vi "Remove Child.vi"(8 "error in (no error)":errorcluster, 10 "Child":refnum<data-value>, 11 "NodeRef In":refnum<data-value>) -> (0 "error out":errorcluster, 2 "Found?":bool, 3 "NodeRef":refnum<data-value>)   [LabVIEW 2020, in "PicoG-ParserLexer.lvlib" / "Node.lvclass"]
doc: "Removes <b>Child</b> from the current node's children list.\n\n<b>Error Codes:</b>\n<b>1556</b>: Uninitialized <b>NodeRef In</b> value, Nodes must be initialized by calling Ctor.\n<b>15</b>: The <b>Child</b> was not found as a child of this node."
uses:
  Node.lvclass
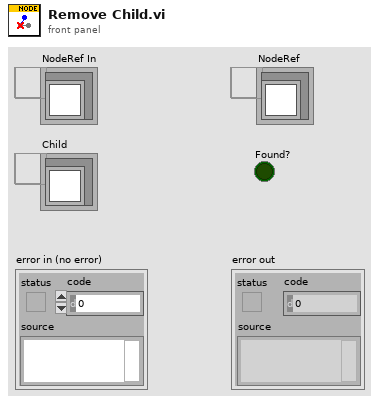
[diagram p1: front panel]
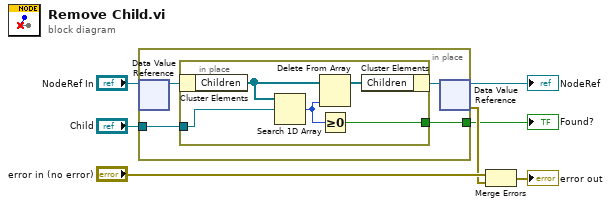
[diagram p0: block diagram]
diagram:
  n1 = in-place {
    in-place-border: "Child" -> [w9]
    in-place-border: [w8] -> w1
    n2 = in-place-dvr #1("NodeRef In") -> (w11:refnum<class "Node.lvclass">)  [unwired: 1 out]
    n3 = in-place {
      in-place-border: w9 -> [w16]
      in-place-border: [w12] -> w8
      n4 = in-place-cluster #2(w11) -> ("Children"=w15:refnum<data-value>[])
      n5 = Search 1D Array(1D array=w15, element=w16) -> (index of element=w13:i32)  [unwired: 1 in]
      n6 = Delete From Array(array=w15, index=w13) -> (array with subset deleted=w14:refnum<data-value>[])  [unwired: 1 in, 1 out]
      n7 = Greater Or Equal To 0?(x=w13) -> (x >= 0?=w12:bool)
      n8 = in-place-cluster #2("Children"=w14) -> (w10:refnum<class "Node.lvclass">)
    }
    n9 = in-place-dvr #1(w10) -> (→"NodeRef":refnum<data-value>, w3:errorcluster)
  }
  "Found?" <- w1
  n10 = Merge Errors("error in (no error)", w3) -> (→"error out":errorcluster)
